vi "test_Basic Waveform Read.vi"(8 "error in (no error)":errorcluster, 11 "DMA Channels Basic Testing in":refnum<class "FPGA Addon DMA Channels Basic System Tests.lvclass">) -> (0 "error out":errorcluster, 3 "DMA Channels Basic Testing out":refnum<class "FPGA Addon DMA Channels Basic System Tests.lvclass">)   [LabVIEW 2020, in "FPGA Addon DMA Channels Basic System Tests.lvclass"]
uses:
  FPGA Addon DMA Channels Basic System Tests.lvclass
  FPGA Addon Test Class/FPGA Addon Test Class.lvclass
panel:
  out "Waveform":waveform(dbl)(graph)
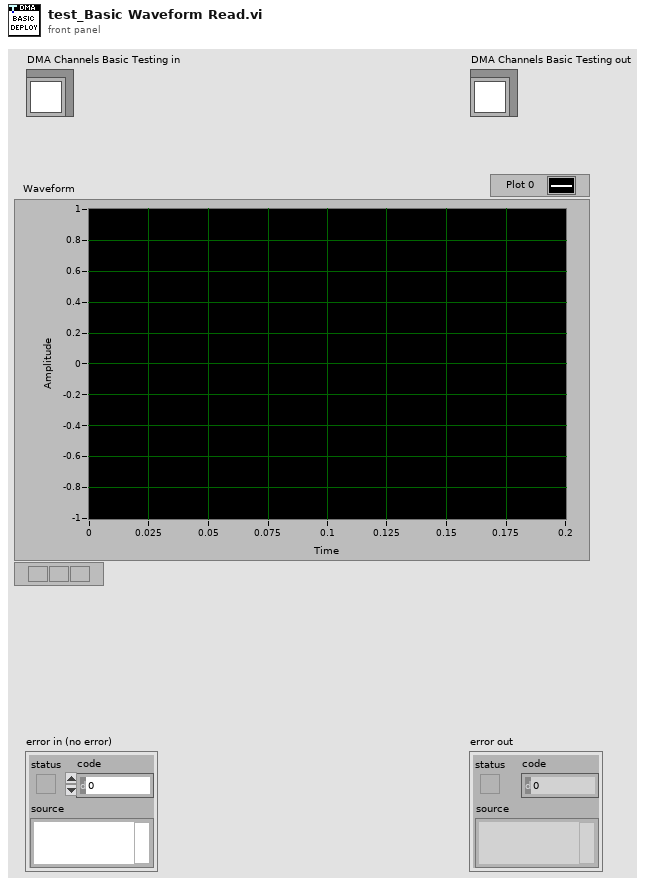
[diagram p1: front panel]
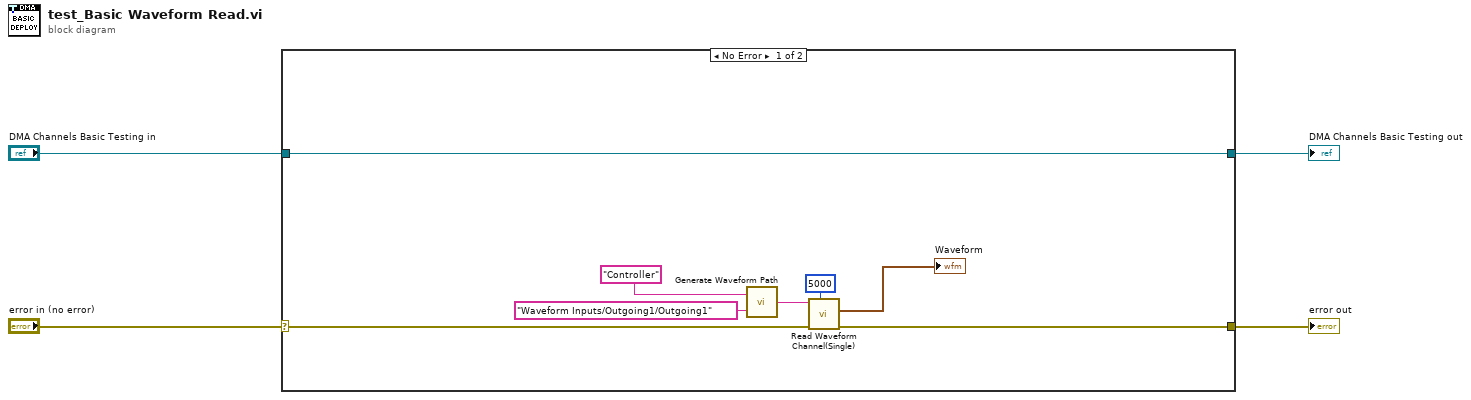
[diagram p0: block diagram]
diagram:
  n1 = case shown="No Error" "error in (no error)" {
    selector: "error in (no error)" -> [w8 w13]
    tunnel: "DMA Channels Basic Testing in" -> [w10 w14]
    tunnel: [w10 w14] -> w3
    tunnel: [w9 w13] -> w2
    frame No Error {
      n2 = call "Generate Waveform Path.vi"("Relative Waveform Path"="Waveform Inputs/Outgoing1/Outgoing1", "Target Name"="Controller") -> ("Waveform Path Out"=w5:string)
      n3 = call "Read Waveform Channel(Single).vi"("Timeout"=5000, "error in (no error)"=w8, "Waveform path in"=w5) -> ("error out"=w9:errorcluster, "Waveform data"=→"Waveform":waveform(dbl))  [unwired: 6 in, 1 out]
    }
    frame Error {
    }
  }
  "error out" <- w2
  "DMA Channels Basic Testing out" <- w3
